vi "UE_Elapsed_Ms.vi"(1 "start_ms":dbl, 2 "now_ms":dbl) -> (0 "elapsed_ms":dbl)   [LabVIEW 2026]
doc: "INTENT: Compute elapsed monotonic milliseconds, caller guarantees now not earlier than start. INPUTS: now_ms (double), start_ms (double). OUTPUTS: elapsed_ms (double). DESIGN CONSTRAINT: Inputs must be monotonic ticks sourced from a common clock domain. REQUIREMENTS: SRS-F-006. No physical hardware side effects. Acceptance requires native LabVIEW compilation and behavioral testing."
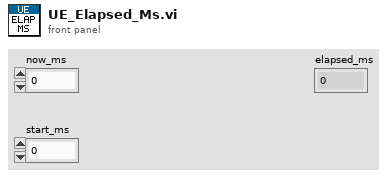
[diagram p1: front panel]
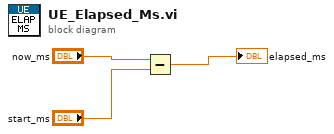
[diagram p0: block diagram]
diagram:
  n1 = Subtract(x="now_ms", y="start_ms") -> (x-y=→"elapsed_ms":dbl)
